vi "Step_On_Timeout.vi"(8 "error in (no error)":errorcluster={"status"=FALSE, "code"=0, "source"="\"\""}, 10 "timer result":string, 11 "StepContext":string) -> (0 "error out":errorcluster={"status"=FALSE, "code"=0, "source"="\"\""}, 2 "status ok":bool, 3 "Retry/Fail/Fault/Stop event":string)   [LabVIEW 2026]
doc: "INTENT: Apply explicit timeout policy. LOGIC: Count bounded retries and branch to correct action; record reason and escalation."
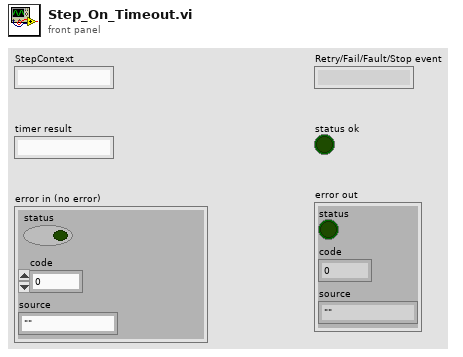
[diagram p1: front panel]
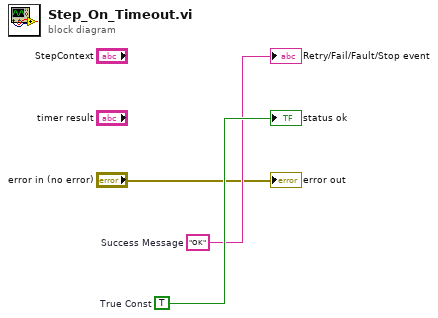
[diagram p0: block diagram]
diagram:
  w3 = TRUE  # True Const
  w2 = "OK"  # Success Message
  "Retry/Fail/Fault/Stop event" <- w2
  "status ok" <- w3
  "error out" <- "error in (no error)"
